vi "DAQ CHx Meas v00 - Sav.vi"(4 "Data File":T1, 6 "Graph":bool, 8 "error in":errorcluster, 9 "DAQ Trigger":T2={"Trig Source"=0, "Digital Trigger"=FALSE, "Trig Edge"=10171, "Pulse Line"=0, "Pulse On Time"=0} {"Pulse Line" items=["/Line0", "/Line1", "/Line2", "/Line3", "/Line4", "/Line5", "/Line6", "/Line7", "/Line8", "/Line9", "/Line10", "/Line11", "/Line12", "/Line13", "/Line14", "/Line15"]; "Trig Edge" items=["Rising"=10280, "Falling"=10171]; "Trig Source" items=["PFI0", "PFI1", "PFI2", "PFI3", "PFI4", "PFI5", "PFI6", "PFI7", "PFI8", "PFI9", "PFI10", "PFI11", "PFI12", "PFI13", "PFI14", "PFI15"]}, 10 "DAQ Timing":T3={"Number of Samples"=100, "Samples Per Second"=1000.0, "Sample Mode"=10178, "Timeout (s)"=10.0} {"Sample Mode" items=["Continuous"=10123, "Finite Sample"=10178, "Hardware Timed Single Point"=12522]}, 11 "DAQ Channel":T4={"Channel"=0, "input terminal configuration"=10106, "Input Range Range"=10.0, "Device"="DAQ1"} {"input terminal configuration" items=["default"=-1, "RSE"=10083, "NRSE"=10078, "Differential"=10106, "Pseudodifferential"=12529]; "Input Range Range" items=["+/-10V"=10.0, "+/-5V"=5.0, "+/-2V"=2.0, "+/-1V"=1.0, "+/-0.5V"=0.5, "+/-0.2V"=0.2, "+/-0.1V"=0.1]; "Channel" items=["0", "1", "2", "3", "4", "5", "6", "7", "8", "9", "10", "11", "12", "13", "14", "15", "16", "17", "16", "19", "20", "21", "22", "23", "24", "25", "26", "27", "28", "29", "30", "31"]}) -> (0 "error out":errorcluster, 3 "Waveform":waveform(dbl))   [LabVIEW 2013]
uses:
  <vilib>/DAQmx/read.llb/DAQmx Read (Analog 1D Wfm NChan NSamp).vi
  <vilib>/DAQmx/create/channels.llb/DAQmx Create Channel (AI-Voltage-Basic).vi
  <vilib>/DAQmx/configure/timing.llb/DAQmx Timing (Sample Clock).vi
  <vilib>/DAQmx/configure/trigger.llb/DAQmx Trigger.vi
  <vilib>/DAQmx/configure/trigger.llb/DAQmx Start Trigger (Digital Edge).vi
  <vilib>/DAQmx/miscellaneous.llb/DAQmx Fill In Error Info.vi
panel:
  in  "Tab Control":enum32{"Setup", "GRaph"}(tab)
  in  "View Settings":bool
  out "Preview Graph":waveform(dbl)(graph)
  out "Physical Channel":string
  out "Sample Mode #":u32
  out "Sample Period":dbl
  out "Sample Interval":dbl
  out "Scope":waveform(dbl)(graph)
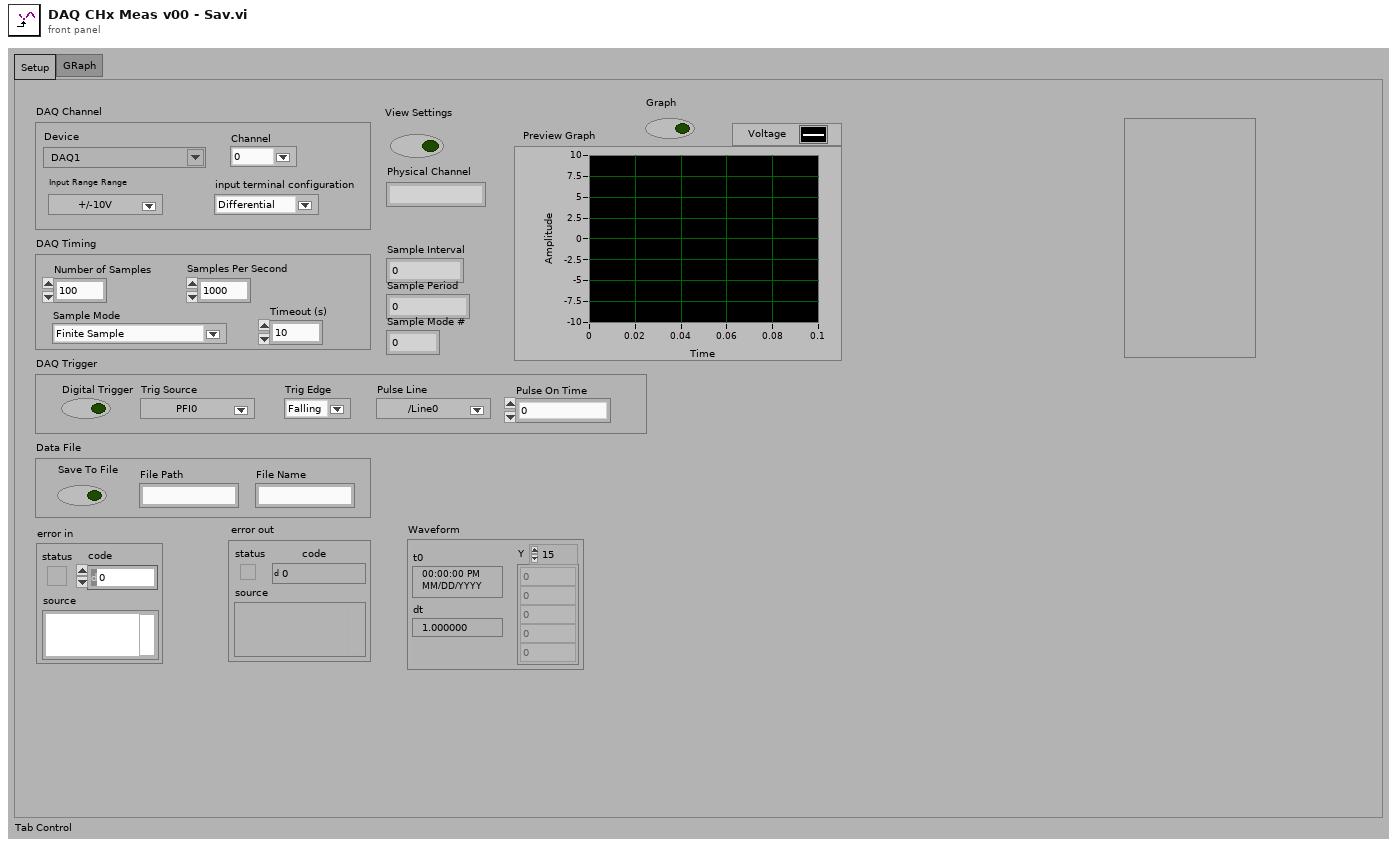
[diagram p1: front panel]
types:
  T1 = cluster{"File Name":string, "File Path":string, "Save To File":bool}
  T2 = cluster{"Trig Source":u16, "Digital Trigger":bool, "Trig Edge":i32, "Pulse Line":u16, "Pulse On Time":u32}
  T3 = cluster{"Number of Samples":u32, "Samples Per Second":dbl, "Sample Mode":i32, "Timeout (s)":dbl}
  T4 = cluster{"Channel":u16, "input terminal configuration":i32, "Input Range Range":dbl, "Device":string}
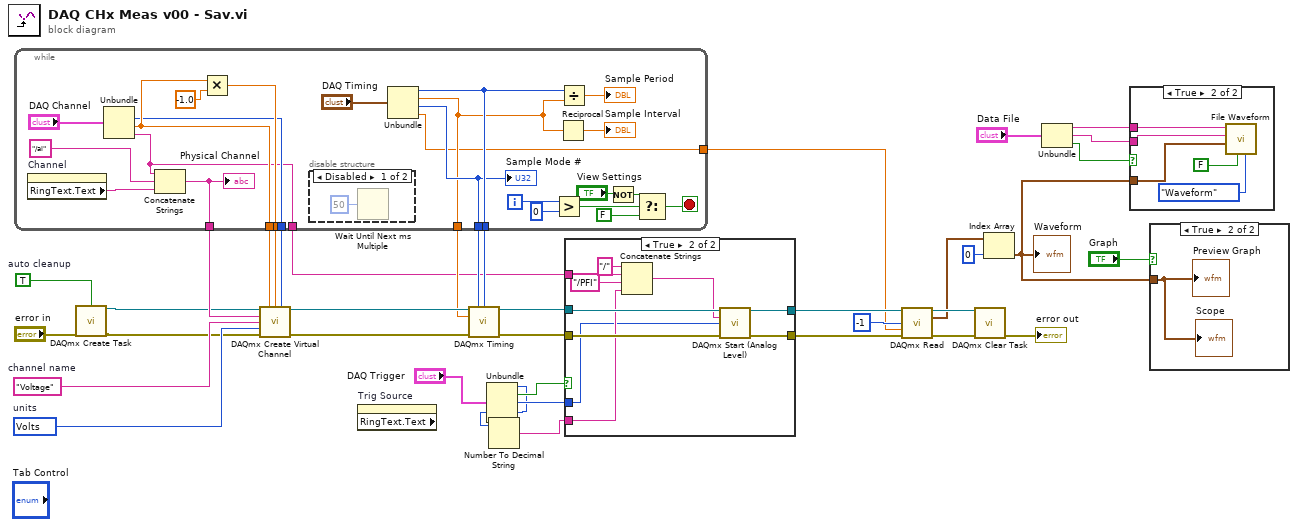
[diagram p0: block diagram]
diagram:
  w36 = 10348 items=["Volts"=10348, "From Custom Scale"=10065]  # units
  w37 = "Voltage"  # channel name
  w8 = TRUE  # auto cleanup
  n1 = while {
    tunnel: [w59] -> w34
    tunnel: [w57] -> w33
    tunnel: [w53] -> w23
    tunnel: [w52] -> w22
    tunnel: [w41] -> w21
    tunnel: [w50] -> w20
    tunnel: [w49] -> w19
    tunnel: [w40] -> w5
    tunnel: [w39] -> w4
    i -> [w45]
    stop <- w44 stop-if-true
    n2 = property on="Channel" class="Ring (strict)"() -> ("RingText.Text"=w60:string)  [unwired: 2 in, 2 out]
    n3 = Unbundle("DAQ Channel") -> ("input terminal configuration"=w52:i32, "Input Range Range"=w53:dbl, "Device"=w39:string)  [unwired: 1 out]
    n4 = Concatenate Strings(w39, "/ai", w60) -> (w59:string)
    "Physical Channel" <- w59
    n5 = Multiply(x=w53, y=-1.0) -> (x*y=w57:dbl)
    n6 = disable-structure shown="Disabled" {
      frame Disabled {
        n7 = Wait Until Next ms Multiple(millisecond multiple=u32 50) -> ()  [unwired: 1 out]
      }
      frame Enabled {
      }
    }
    n8 = Unbundle("DAQ Timing") -> ("Number of Samples"=w50:u32, "Samples Per Second"=w41:dbl, "Sample Mode"=w49:i32, "Timeout (s)"=w40:dbl)
    "Sample Mode #" <- w49
    n9 = Greater?(x=w45, y=0) -> (0:w47:bool)
    n10 = Reciprocal(x=w41) -> (1/x=→"Sample Interval":dbl)
    n11 = Divide(x=w50, y=w41) -> (x/y=→"Sample Period":dbl)
    n12 = Not(x="View Settings") -> (.not. x?=w43:bool)
    n13 = Select(t=w43, s=w47, f=FALSE) -> (s? t:f=w44:bool)
  }
  n14 = call <vilib>:"DAQmx Create Task.vi"("auto cleanup"=w8, "error in"="error in") -> ("task out"=w10:refnum<k21>, "error out"=w9:errorcluster)  [unwired: 12 in]
  n15 = call-poly <vilib>:"DAQmx Create Virtual Channel.vi"("task in"=w10, "maximum value"=w23, "minimum value"=w33, "input terminal configuration"=w22, "physical channels"=w34, "name to assign"=w37, "units"=w36, "error in"=w9) -> ("task out"=w35:refnum<k21>, "error out"=w38:errorcluster)  [unwired: 6 in]
  n16 = property on="Trig Source" class="Ring (strict)" props=["RingText", "Text"]() -> ()  [unwired: 2 in, 3 out]
  n17 = call-poly <vilib>:"DAQmx Timing.vi"("task/channels in"=w35, "sample mode"=w19, "samples per channel"=w20, "rate"=w21, "error in"=w38) -> ("task out"=w26:refnum<k21>, "error out"=w12:errorcluster)  [unwired: 9 in]
  n18 = Unbundle("DAQ Trigger") -> ("Trig Source"=w1:u16, "Digital Trigger"=w2:bool, "Trig Edge"=w17:i32)  [unwired: 2 out]
  n19 = Number To Decimal String(number=w1) -> (decimal integer string=w3:string)  [unwired: 1 in]
  n20 = case shown="True" w2 {
    tunnel: w12 -> [w64 w73]
    tunnel: [w64 w72] -> w27
    tunnel: w26 -> [w63 w74]
    tunnel: [w63 w71] -> w25
    tunnel: w17 -> [_ w67]
    tunnel: w4 -> [_ w70]
    tunnel: w3 -> [_ w69]
    frame False {
    }
    frame True {
      n21 = Concatenate Strings("/" ("string"), w70, "/PFI" ("string"), w69) -> (w66:string)
      n22 = call-poly "DAQmx Start (Analog Level).vi"("task/channels in"=w74, "source"=w66, "edge"=w67, "error in"=w73) -> ("task out"=w71:refnum<k21>, "error out"=w72:errorcluster)  [unwired: 10 in]
    }
  }
  n23 = call-poly <vilib>:"DAQmx Read.vi"("task/channels in"=w25, "number of samples per channel"=-1, "timeout"=w5, "error in"=w27) -> ("task out"=w31:refnum<k21>, "data"=w30:waveform(dbl)[], "error out"=w24:errorcluster)  [unwired: 9 in]
  n24 = call <vilib>:"DAQmx Clear Task.vi"("task in"=w31, "error in"=w24) -> ("error out"=→"error out":errorcluster)  [unwired: 13 in]
  n25 = Index Array(array=w30, index=0) -> (element=w32:waveform(dbl))
  "Waveform" <- w32
  n26 = Unbundle("Data File") -> ("File Name"=w15:string, "File Path"=w14:string, "Save To File"=w13:bool)
  n27 = case shown="True" w13 {
    tunnel: w32 -> [_ w79]
    tunnel: w15 -> [_ w77]
    tunnel: w14 -> [_ w76]
    frame False {
    }
    frame True {
      n28 = call "File Waveform.vi"("File Format"=enum16{"Spreadsheet", "Waveform", ""}."Waveform", "Append Time"=FALSE, "waveform"=w79, "File Path"=w76, "File Name"=w77) -> ()  [unwired: 4 in, 3 out]
    }
  }
  n29 = case shown="True" "Graph" {
    tunnel: w32 -> [_ w80]
    frame False {
    }
    frame True {
      "Scope" <- w80
      "Preview Graph" <- w80
    }
  }
